vi "Obtain_Message_Queue.vi"(8 "error in (no error)":errorcluster={"status"=FALSE, "code"=0, "source"="\"\""}) -> (0 "error out":errorcluster, 3 "Message Queue":refnum<queue>)   [LabVIEW 2026]
doc: "Create a queue with Message payload."
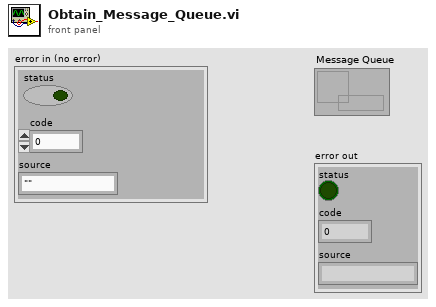
[diagram p1: front panel]
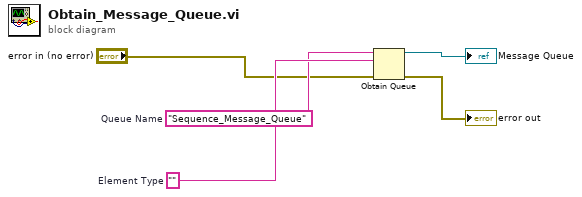
[diagram p0: block diagram]
diagram:
  w3 = ""  # Element Type
  w2 = "Sequence_Message_Queue"  # Queue Name
  n1 = Obtain Queue(name (unnamed)=w2, element data type=w3, error in (no error)="error in (no error)") -> (queue out=→"Message Queue":refnum<queue>, error out=→"error out":errorcluster)  [unwired: 2 in, 1 out]
